vi "ZMQ.Connect.vi"(7 "socket type":T1, 8 "error in (no error)":errorcluster, 9 "port":u16, 10 "address":string, 11 "RemoteControl.ZMQ in":refnum<class "RemoteControl.ZMQ.lvclass">) -> (0 "error out":errorcluster, 3 "RemoteControl.ZMQ out":refnum<class "RemoteControl.ZMQ.lvclass">)   [LabVIEW 2019, in "RemoteControl.ZMQ.lvlib" / "RemoteControl.ZMQ.lvclass"]
uses:
  RemoteControl.ZMQ.lvclass
  <vilib>/addons/zeromq/socket_type.ctl
  RemoteControl.ZMQ.lvclass/RemoteControl.ZMQ.ctl
  <vilib>/addons/zeromq/zmq_socket.lvclass
  <vilib>/addons/zeromq/zmq_context.lvclass
  <vilib>/addons/zeromq/zeromq.lvlib
  ZMQ.ContextManager/ZMQ.ContextManager.lvlib
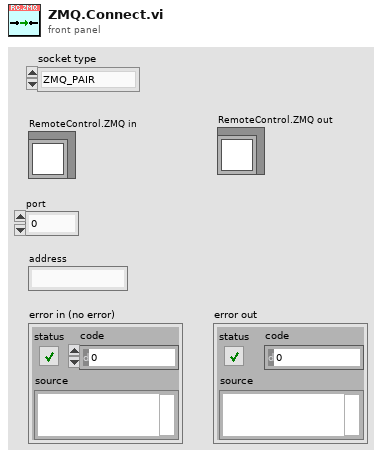
[diagram p1: front panel]
types:
  T1 = typedef "zeromq.lvlib/socket_type.ctl" = enum8{"ZMQ_PAIR", "ZMQ_PUB", "ZMQ_SUB", "ZMQ_REQ", "ZMQ_REP", "ZMQ_DEALER", "ZMQ_ROUTER", "ZMQ_PULL", "ZMQ_PUSH", "ZMQ_XPUB", "ZMQ_XSUB", "ZMQ_STREAM", "ZMQ_SERVER", "ZMQ_CLIENT", "ZMQ_RADIO", "ZMQ_DISH", "ZMQ_GATHER", "ZMQ_SCATTER", "ZMQ_DGRAM"}
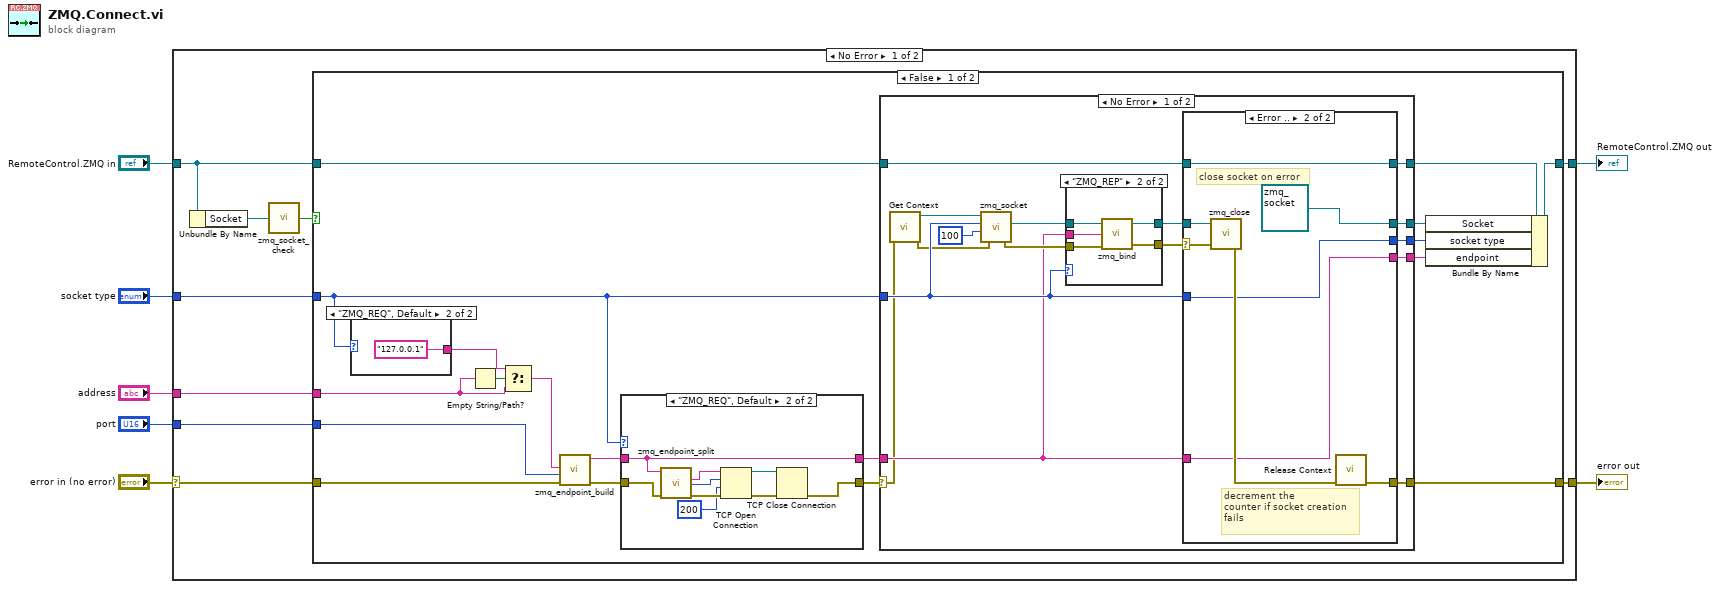
[diagram p0: block diagram]
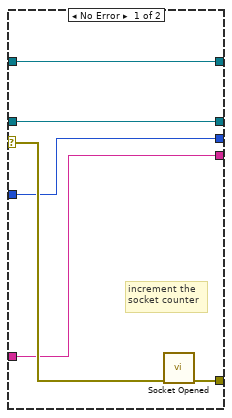
[diagram p3: hidden frame]
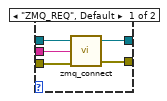
[diagram p4: hidden frame]
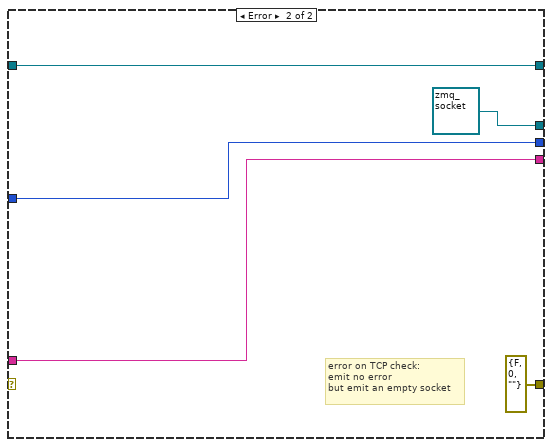
[diagram p5: hidden frame]
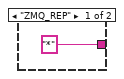
[diagram p6: hidden frame]
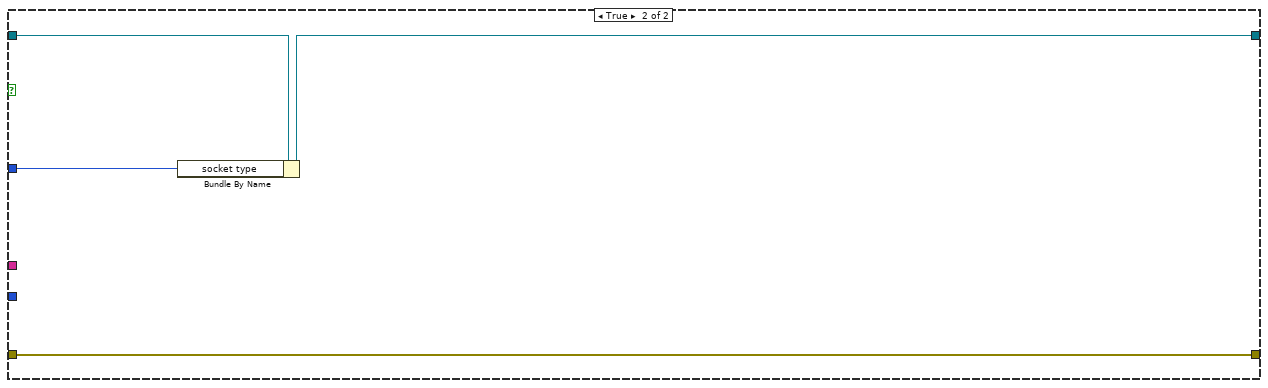
[diagram p7: hidden frame]
diagram:
  n1 = case shown="No Error" "error in (no error)" {
    selector: "error in (no error)" -> [w10 w98]
    tunnel: "RemoteControl.ZMQ in" -> [w14 w97]
    tunnel: [w13 w98] -> w2
    tunnel: [w12 w97] -> w3
    tunnel: "address" -> [w11 _]
    tunnel: "port" -> [w9 _]
    tunnel: "socket type" -> [w8 _]
    frame No Error {
      n2 = Unbundle By Name(w14) -> ("Socket"=w15:refnum<class "zmq_socket.lvclass">)
      n3 = call <vilib>:"zmq_socket_check.vi"("socket in"=w15) -> ("valid?"=w16:bool)
      n4 = case shown="False" w16 {
        tunnel: w8 -> [w24 w95]
        tunnel: w14 -> [w29 w94]
        tunnel: [w19 w93] -> w12
        tunnel: w10 -> [w32 w96]
        tunnel: [w30 w96] -> w13
        tunnel: w11 -> [w31 _]
        tunnel: w9 -> [w28 _]
        frame False {
          n5 = case shown="\"ZMQ_REQ\", Default" w24 {
            tunnel: ["*" ("t") "127.0.0.1" ("t")] -> w33
            frame "ZMQ_REP" {
            }
            frame "ZMQ_REQ", Default {
            }
          }
          n6 = Empty String/Path?(string/path=w31) -> (empty?=w34:bool)
          n7 = Select(t=w33, s=w34, f=w31) -> (s? t:f=w27:string)
          n8 = call <vilib>:"zmq_endpoint_build.vi"("error in"=w32, "port"=w28, "address"=w27) -> ("error out"=w26:errorcluster, "endpoint"=w25:string)  [unwired: 2 in, 1 out]
          n9 = case shown="\"ZMQ_REQ\", Default" w24 {
            tunnel: w26 -> [w35 w41]
            tunnel: w25 -> [w36 w39]
            tunnel: [w36 w39] -> w23
            tunnel: [w35 w38] -> w22
            frame "ZMQ_REP" {
            }
            frame "ZMQ_REQ", Default {
              n10 = call <vilib>:"zmq_endpoint_split.vi"("error in"=w41, "endpoint"=w39) -> ("error out"=w43:errorcluster, "port"=w42:u16, "address"=w40:string)  [unwired: 2 in, 1 out]
              n11 = TCP Open Connection(address=w40, remote port or service name=w42, timeout ms (60000)=200, error in (no error)=w43) -> (connection ID=w44:refnum<k5>, error out=w45:errorcluster)  [unwired: 1 in]
              n12 = TCP Close Connection(connection ID=w44, error in (no error)=w45) -> (error out=w38:errorcluster)  [unwired: 1 in, 1 out]
            }
          }
          n13 = case shown="No Error" w22 {
            selector: w22 -> [w50 _]
            tunnel: [w58 w89] -> w20
            tunnel: [w57 errorcluster {"status"=FALSE, "code"=0, "source"=""} ("error out")] -> w30
            tunnel: w29 -> [w55 w89]
            tunnel: w24 -> [w52 w87]
            tunnel: w23 -> [w51 w86]
            tunnel: [w48 refnum<class "zmq_socket.lvclass"> refnum ("socket out")] -> w21
            tunnel: [w47 w87] -> w18
            tunnel: [w46 w86] -> w17
            frame No Error {
              n14 = call "Get Context.vi"("error in"=w50) -> ("error out"=w49:errorcluster, "context"=w60:refnum<class "zmq_context.lvclass">)  [unwired: 9 in]
              n15 = call <vilib>:"zmq_socket.vi"("error in"=w49, "linger (ms)"=100, "socket type"=w52, "context in"=w60) -> ("error out"=w53:errorcluster, "socket out"=w54:refnum<class "zmq_socket.lvclass">)  [unwired: 1 in, 1 out]
              n16 = case shown="\"ZMQ_REP\"" w52 {
                tunnel: w54 -> [w77 w85]
                tunnel: [w80 w84] -> w59
                tunnel: w51 -> [w79 w83]
                tunnel: [w78 w82] -> w56
                tunnel: w53 -> [w76 w81]
                frame "ZMQ_REQ", Default {
                  n17 = call <vilib>:"zmq_connect.vi"("error in"=w76, "endpoint"=w79, "socket in"=w77) -> ("error out"=w78:errorcluster, "socket out"=w80:refnum<class "zmq_socket.lvclass">)  [unwired: 1 in]
                }
                frame "ZMQ_REP" {
                  n18 = call <vilib>:"zmq_bind.vi"("error in"=w81, "endpoint"=w83, "socket in"=w85) -> ("error out"=w82:errorcluster, "socket out"=w84:refnum<class "zmq_socket.lvclass">)  [unwired: 1 in]
                }
              }
              n19 = case shown="Error .." w56 {
                selector: w56 -> [w66 w72]
                tunnel: w59 -> [w64 w73]
                tunnel: w55 -> [w65 w75]
                tunnel: [w65 w75] -> w58
                tunnel: w52 -> [w63 w70]
                tunnel: w51 -> [w62 w68]
                tunnel: [w67 w74] -> w57
                tunnel: [w64 refnum<class "zmq_socket.lvclass"> refnum ("socket out")] -> w48
                tunnel: [w63 w70] -> w47
                tunnel: [w62 w68] -> w46
                frame No Error {
                  # "increment the \nsocket counter"
                  n20 = call "Socket Opened.vi"("error in"=w66) -> ("error out"=w67:errorcluster)  [unwired: 10 in]
                }
                frame Error {
                  # "close socket on error"
                  # "decrement the \ncounter if socket creation\nfails"
                  n21 = call <vilib>:"zmq_close.vi"("error in"=w72, "socket"=w73) -> ("error out"=w71:errorcluster)  [unwired: 3 in]
                  n22 = call "Release Context.vi"("error in"=w71) -> ("error out"=w74:errorcluster)  [unwired: 9 in, 1 out]
                }
              }
            }
            frame Error {
              # "error on TCP check:\nemit no error\nbut emit an empty socket"
            }
          }
          n23 = Bundle By Name(cluster=w20, "Socket"=w21, "socket type"=w18, "endpoint"=w17) -> (w19:refnum<class "RemoteControl.ZMQ.lvclass">)
        }
        frame True {
          n24 = Bundle By Name(cluster=w94, "socket type"=w95) -> (w93:refnum<class "RemoteControl.ZMQ.lvclass">)
        }
      }
    }
    frame Error {
    }
  }
  "RemoteControl.ZMQ out" <- w3
  "error out" <- w2
